vi "reset SA Device.vi"(8 "error in (no error)":errorcluster, 11 "FSV-40N in":refnum<class "FSV-40N.lvclass">) -> (0 "error out":errorcluster, 3 "FSV-40N out":refnum<class "FSV-40N.lvclass">)   [LabVIEW 2023, in "Spectrum Analyzer.lvlib" / "FSV-40N.lvclass"]
uses:
  FSV-40N.lvclass
  FSV-40N.lvclass/FSV-40N.ctl
  TYPE DEFINITION/TYPE Marker Control Mode.ctl
  Spectrum Analyzer.lvlib
  TYPE DEFINITION/TYPE Marker Type Map.ctl
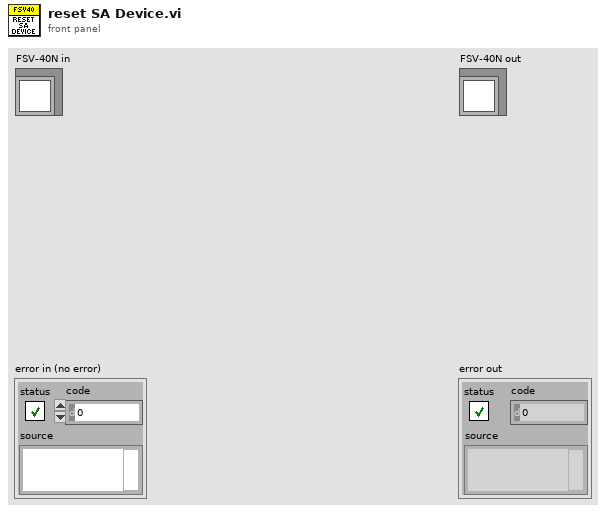
[diagram p1: front panel]
types:
  T1 = typedef "Spectrum Analyzer.lvlib/TYPE Marker Type Map.ctl" = map{i32, T2}
  T2 = typedef "Spectrum Analyzer.lvlib/TYPE Marker Control Mode.ctl" = enum16{"Normal", "Delta", "Off"}
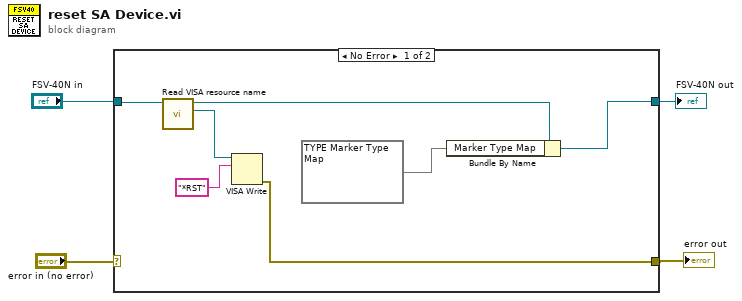
[diagram p0: block diagram]
diagram:
  n1 = case shown="No Error" "error in (no error)" {
    selector: "error in (no error)" -> [_ w12]
    tunnel: [w8 w12] -> w3
    tunnel: "FSV-40N in" -> [w11 w13]
    tunnel: [w5 w13] -> w1
    frame No Error {
      n2 = call "Read VISA resource name.vi"("FSV-40N in"=w11) -> ("VISA resource name"=w10:refnum<visa-resource-name>, "FSV-40N out"=w7:refnum<class "FSV-40N.lvclass">)  [unwired: 8 in, 1 out]
      n3 = VISA Write(VISA resource name=w10, write buffer="*RST") -> (error out=w8:errorcluster)  [unwired: 1 in, 2 out]
      n4 = Bundle By Name(cluster=w7, "Marker Type Map"=T1 {}) -> (w5:refnum<class "FSV-40N.lvclass">)
    }
    frame Error {
    }
  }
  "error out" <- w3
  "FSV-40N out" <- w1
